vi "Get OOB gRPC Port.vi"(8 "error in (no error)":errorcluster) -> (0 "error out":errorcluster, 3 "OOB gRPC Port":i32)   [LabVIEW 2025, in "I2C Bus Monitor.lvclass"]
uses:
  I2C Bus Monitor.lvclass
  I2C Bus Monitor.lvclass/I2C Bus Monitor.ctl
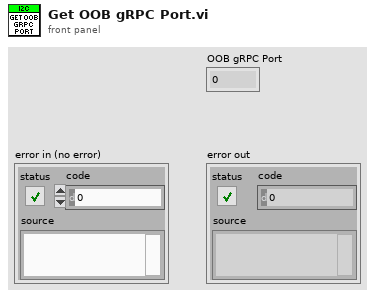
[diagram p1: front panel]
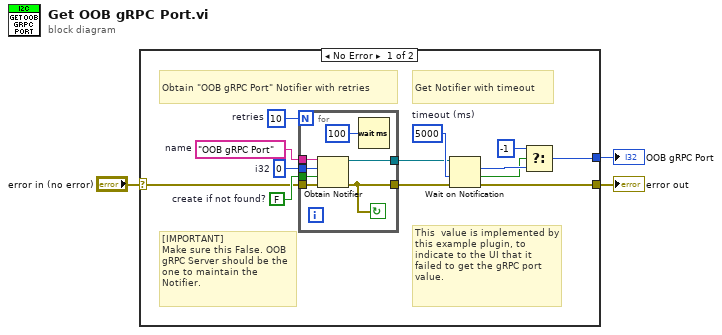
[diagram p0: block diagram]
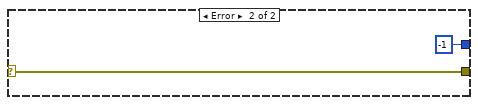
[diagram p2: hidden frame]
diagram:
  n1 = case shown="No Error" "error in (no error)" {
    selector: "error in (no error)" -> [w9 w25]
    tunnel: [w12 -1 ("i32")] -> w3
    tunnel: [w11 w25] -> w2
    frame No Error {
      w16 = FALSE  # create if not found?
      w8 = 0  # i32
      w10 = "OOB gRPC Port"  # name
      w7 = 10  # retries
      w6 = 5000  # timeout (ms)
      # "This  value is implemented by this example plugin, to indicate to the UI that it failed to get the gRPC port value."
      # "[IMPORTANT] \nMake sure this False. OOB gRPC Server should be the one to maintain the Notifier."
      # "Obtain \"OOB gRPC Port\" Notifier with retries"
      # "Get Notifier with timeout"
      n2 = for {
        N: w7 -> [_]
        tunnel: [w21] -> w4
        tunnel: [w23] -> w5
        tunnel: w10 -> [w20]
        tunnel: w8 -> [w19]
        tunnel: w9 -> [w18]
        tunnel: w16 -> [w17]
        stop <- w21 continue-if-true
        n3 = Obtain Notifier(name (unnamed)=w20, notification data type=w19, create if not found? (T)=w17, error in (no error)=w18) -> (notifier out=w23:refnum<notifier>, error out=w21:errorcluster)  [unwired: 1 out]
        n4 = Wait (ms)(milliseconds to wait=u32 100) -> ()  [unwired: 1 out]
      }
      n5 = Wait on Notification(notifier=w5, timeout in ms (-1)=w6, error in (no error)=w4) -> (notification=w14:i32, timed out?=w13:bool, error out=w11:errorcluster)  [unwired: 1 in, 1 out]
      n6 = Select(t=-1, s=w13, f=w14) -> (s? t:f=w12:i32)
    }
    frame Error {
    }
  }
  "OOB gRPC Port" <- w3
  "error out" <- w2
